vi "SetValueByItemName.vi"(0 "VI Reference In":refnum<vi>, 2 "delimiter (>>)":string=">>", 5 "Control Path":string, 7 "Item Name":string, 9 "Occurrence":i32=1, 11 "Error In":errorcluster) -> (4 "VI Reference Out":refnum<vi>, 15 "Error Out":errorcluster)   [LabVIEW 2016, in "Drona.lvlib" / "ControlValue.lvlib" / "StimulusListbox.lvlib"]
doc: "Sets value(signaling) for the listbox control whose item name is specified with its occurrence. Set the value as 1 in occurrence to select the first occurrence of an item. \n\nThe input control name is given as a string , incase of path, use delimiters inbetween the path."
uses:
  StimulusListbox.lvlib
  <userlib>/_OpenG.lib/array/array.llb/Search 1D Array (String)__ogtk.vi
  <vilib>/Utility/error.llb/Error Cluster From Error Code.vi
  <vilib>/ErrorRing/Error Ring.xnode
  Drona.lvlib
  Get/GetControlRef/GetControlRef.lvlib
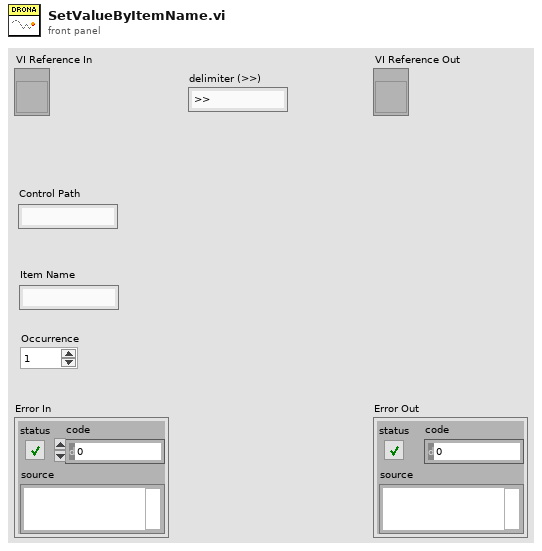
[diagram p1: front panel]
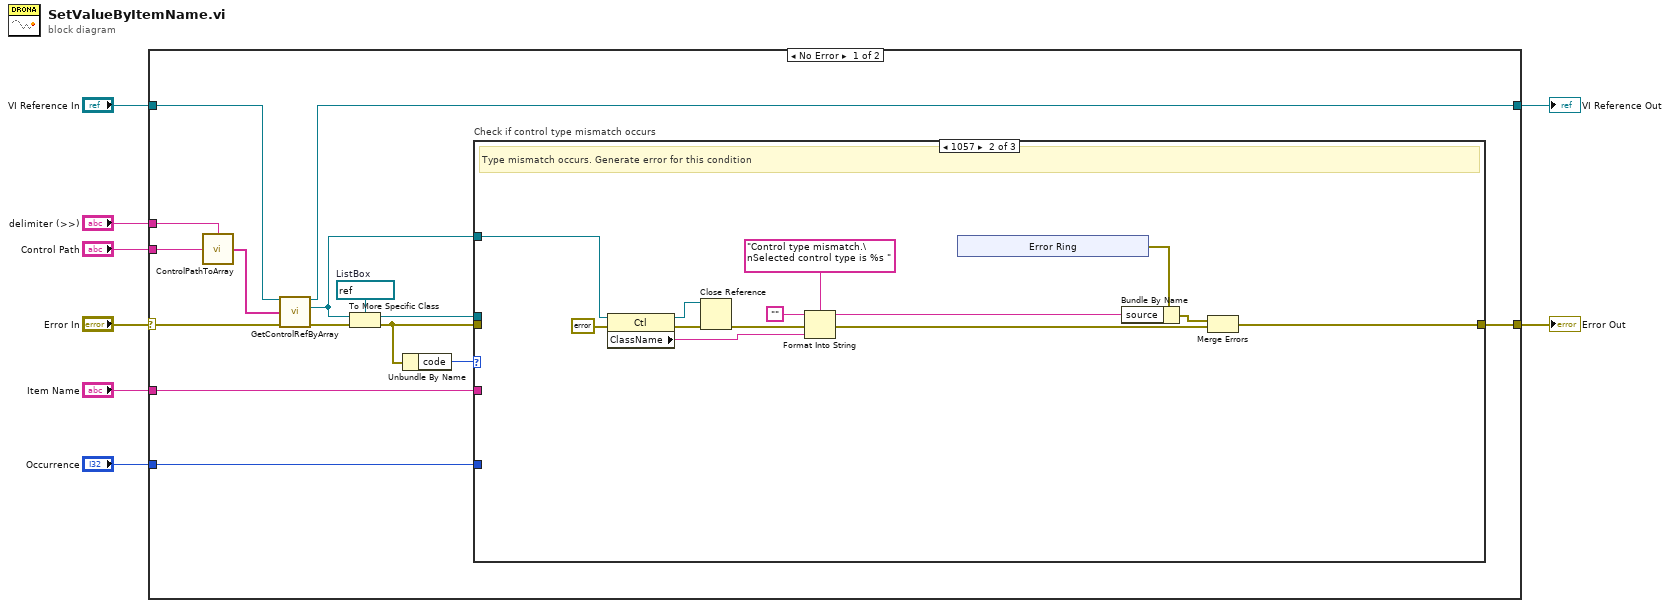
[diagram p0: block diagram]
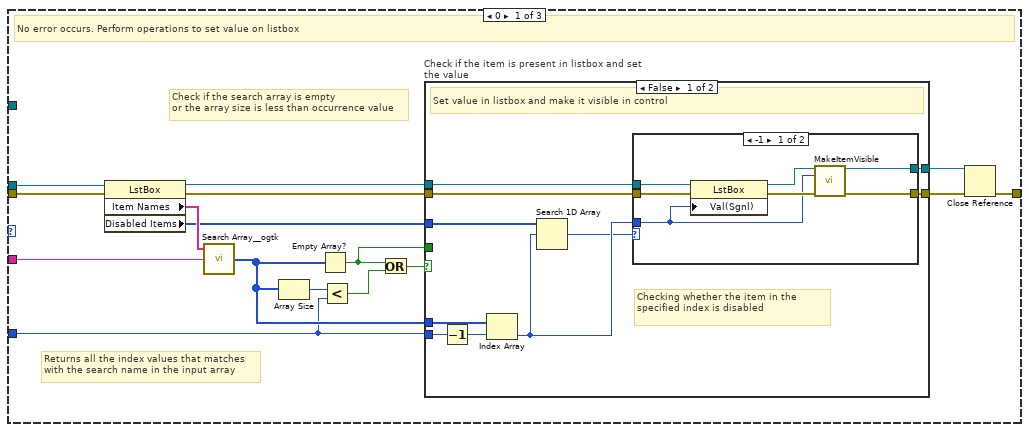
[diagram p2: hidden frame]
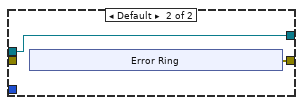
[diagram p3: hidden frame]
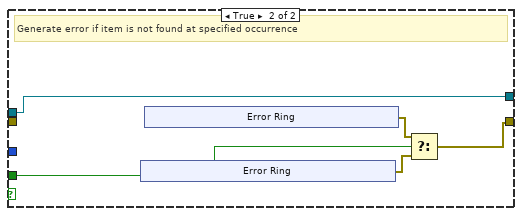
[diagram p4: hidden frame]
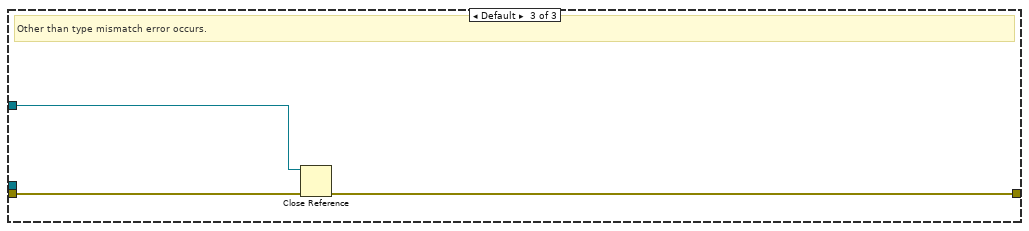
[diagram p5: hidden frame]
diagram:
  n1 = case shown="No Error" "Error In" {
    selector: "Error In" -> [w18 w101]
    tunnel: [w19 w101] -> w7
    tunnel: "VI Reference In" -> [w17 w100]
    tunnel: "Control Path" -> [w21 _]
    tunnel: [w14 w100] -> w4
    tunnel: "delimiter (>>)" -> [w20 _]
    tunnel: "Item Name" -> [w13 _]
    tunnel: "Occurrence" -> [w12 _]
    frame No Error {
      w23 = refnum<vi> refnum  # ListBox
      n2 = call "ControlPathToArray.vi"("Control Name"=w21, "delimiter (>>)"=w20) -> ("Control Path"=w16:string[])
      n3 = call "GetControlRefByArray.vi"("VI Reference In"=w17, "Control Path"=w16, "error In"=w18) -> ("VI Reference Out"=w14:refnum<vi>, "Ctl Refnum"=w9:refnum<vi>, "error out"=w15:errorcluster)  [unwired: 10 in]
      n4 = To More Specific Class(target class=w23, reference=w9, error in=w15) -> (specific class reference=w22:refnum<vi>, error out=w11:errorcluster)
      n5 = Unbundle By Name(w11) -> ("code"=w10:i32)
      n6 = case "Check if control type mismatch occurs" shown="1057" w10 {
        tunnel: w11 -> [w39 _ w99]
        tunnel: w22 -> [w38 _ _]
        tunnel: [w37 w79 w98] -> w19
        tunnel: w13 -> [w33 _ _]
        tunnel: w12 -> [w28 _ _]
        tunnel: w9 -> [_ w80 w97]
        frame 0 {
          # "Check if the search array is empty \nor the array size is less than occurrence value"
          # "Returns all the index values that matches\nwith the search name in the input array"
          # "No error occurs. Perform operations to set value on listbox"
          n7 = property class="LstBox"(reference=w38, error in=w39) -> (reference out=w26:refnum<vi>, error out=w27:errorcluster, "Item Names"=w34:string[], "Disabled Items"=w24:i32[])
          n8 = call-poly <userlib>:"Search Array__ogtk.vi"("Array"=w34, "Element Data"=w33) -> ("Indices of Elements"=w29:i32[])  [unwired: 7 in]
          n9 = Array Size(array=w29) -> (size(s)=w32:i32)
          n10 = Empty Array?(array=w29) -> (empty?=w25:bool)
          n11 = Less?(x=w32, y=w28) -> (x < y?=w31:bool)
          n12 = Or(x=w25, y=w31) -> (x .or. y?=w30:bool)
          n13 = case "Check if the item is present in listbox and set the value" shown="False" w30 {
            tunnel: [w49 w68] -> w36
            tunnel: [w48 w67] -> w35
            tunnel: w29 -> [w47 _]
            tunnel: w28 -> [w46 _]
            tunnel: w27 -> [w44 _]
            tunnel: w26 -> [w43 w67]
            tunnel: w25 -> [_ w66]
            tunnel: w24 -> [w42 _]
            frame False {
              # "Checking whether the item in the specified index is disabled"
              # "Set value in listbox and make it visible in control"
              n14 = Decrement(x=w46) -> (x-1=w45:i32)
              n15 = Index Array(array=w47, index=w45) -> (element=w41:i32)
              n16 = Search 1D Array(1D array=w42, element=w41) -> (index of element=w40:i32)  [unwired: 1 in]
              n17 = case shown="-1" w40 {
                tunnel: [w55 w57] -> w49
                tunnel: [w53 w58] -> w48
                tunnel: w41 -> [w52 _]
                tunnel: w44 -> [w51 _]
                tunnel: w43 -> [w50 w58]
                frame -1 {
                  n18 = property class="LstBox"(reference=w50, error in=w51, "Val(Sgnl)"=w52) -> (reference out=w54:refnum<vi>, error out=w56:errorcluster)
                  n19 = call "MakeItemVisible.vi"("ListBox Ref In"=w54, "Item Index"=w52, "Error In"=w56) -> ("ListBox Ref Out"=w53:refnum<vi>, "Error Out"=w55:errorcluster)  [unwired: 11 in]
                }
                frame Default {
                  n20 = xnode "Error Ring"() -> ("error out"=w57:errorcluster)
                }
              }
            }
            frame True {
              # "Generate error if item is not found at specified occurrence"
              n21 = xnode "Error Ring"() -> ("error out"=w64:errorcluster)
              n22 = xnode "Error Ring"() -> ("error out"=w65:errorcluster)
              n23 = Select(t=w65, s=w66, f=w64) -> (s? t:f=w68:errorcluster)
            }
          }
          n24 = Close Reference(reference=w35, error in (no error)=w36) -> (error out=w37:errorcluster)
        }
        frame 1057 {
          # "Type mismatch occurs. Generate error for this condition"
          n25 = property class="Ctl"(reference=w80, error in=errorcluster {"status"=FALSE, "code"=0, "source"=""} ("error out")) -> (reference out=w81:refnum<vi>, error out=w91:errorcluster, "ClassName"=w88:string)
          n26 = Close Reference(reference=w81, error in (no error)=w91) -> (error out=w82:errorcluster)
          n27 = Format Into String(format string="Control type mismatch.\nSelected control type is %s ", initial string="", error in=w82, w88) -> (resulting string=w85:string, error out=w83:errorcluster)
          n28 = xnode "Error Ring"() -> ("error out"=w86:errorcluster)
          n29 = Bundle By Name(cluster=w86, "source"=w85) -> (w84:errorcluster)
          n30 = Merge Errors(w84, w83) -> (w79:errorcluster)
        }
        frame Default {
          # "Other than type mismatch error occurs."
          n31 = Close Reference(reference=w97, error in (no error)=w99) -> (error out=w98:errorcluster)
        }
      }
    }
    frame Error {
    }
  }
  "Error Out" <- w7
  "VI Reference Out" <- w4
